vi "Own20261012_GetInvokeTerminals.vi"() -> ()   [LabVIEW 2024]
panel:
  out "error out":errorcluster caption="错误输出"
  out "output_terminal_ids":refnum<vi>[](array[refnum])
  out "input_terminal_ids":refnum<vi>[](array[refnum])
  in  "invoke_id":u32
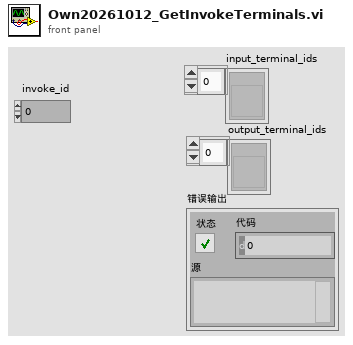
[diagram p1: front panel]
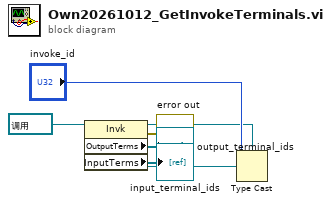
[diagram p0: block diagram]
diagram:
  n1 = Type Cast(type=refnum<vi> refnum ("引用"), x="invoke_id") -> (*(type *) &x=w4:refnum<vi>)
  n2 = property class="Invk"(reference=w4) -> (error out=→"error out":errorcluster, "OutputTerms"=→"output_terminal_ids":refnum<vi>[], "InputTerms"=→"input_terminal_ids":refnum<vi>[])  [unwired: 1 in, 1 out]
